vi "Get_SglVar_Value.vi"(8 "error in (no error)":errorcluster, 11 "muExpr in":refnum<class "mupExpr.lvclass">) -> (0 "error out":errorcluster, 2 "Value":dbl, 3 "muExpr out":refnum<class "mupExpr.lvclass">)   [LabVIEW 2018, in "mupExpr.lvclass"]
doc: "Return the expression's single variable value."
uses:
  mupExpr.lvclass
  mupExpr.lvclass/mupExpr.ctl
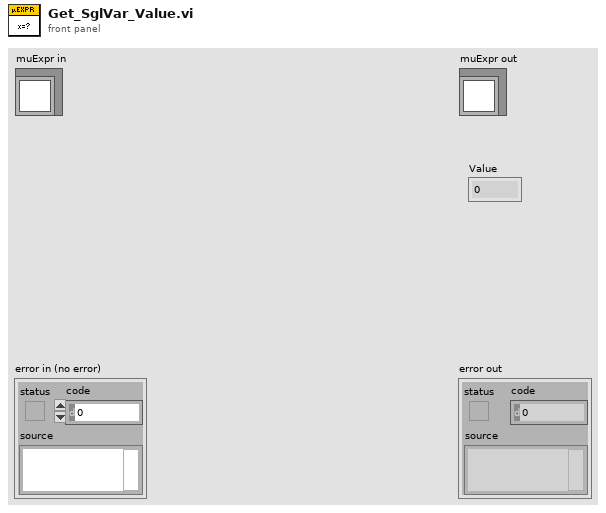
[diagram p1: front panel]
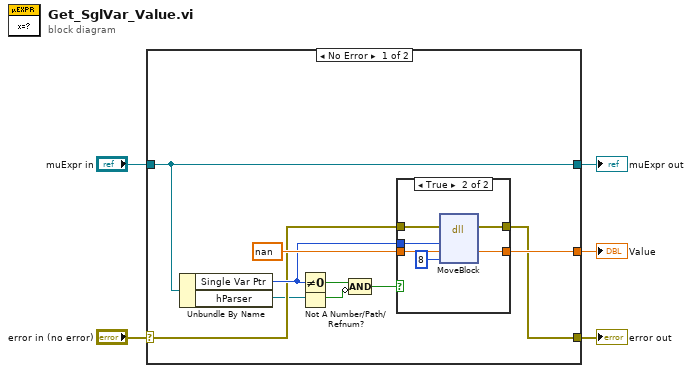
[diagram p0: block diagram]
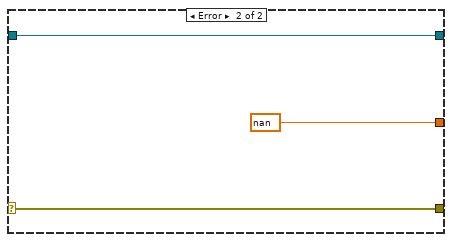
[diagram p3: hidden frame]
diagram:
  n1 = case shown="No Error" "error in (no error)" {
    selector: "error in (no error)" -> [w12 w26]
    tunnel: [w11 w26] -> w4
    tunnel: [w6 w25] -> w2
    tunnel: "muExpr in" -> [w6 w25]
    tunnel: [w15 nan ("pd")] -> w1
    frame No Error {
      n2 = Unbundle By Name(w6) -> ("Single Var Ptr"=w13:u64, "hParser"=w7:refnum<data-value>)
      n3 = Not Equal To 0?(x=w13) -> (x != 0?=w9:bool)
      n4 = Not A Number/Path/Refnum?(number/path/refnum=w7) -> (NaN/Path/Refnum?=w10:bool)
      n5 = Compound Arithmetic op=AND(w9, invert w10) -> (w8:bool)
      n6 = case shown="True" w8 {
        tunnel: nan ("pd") -> [w16 w22]
        tunnel: w12 -> [w17 w21]
        tunnel: [w17 w20] -> w11
        tunnel: w13 -> [_ w19]
        tunnel: [w16 w18] -> w15
        frame False {
        }
        frame True {
          n7 = dll-call lib="LabVIEW" fn="MoveBlock"(error in=w21, "ps"=w19, "pd"=w22, "size"=8) -> (error out=w20:errorcluster, "pd"=w18:dbl)  [unwired: 5 in, 1 out]
        }
      }
    }
    frame Error {
    }
  }
  "error out" <- w4
  "muExpr out" <- w2
  "Value" <- w1
